vi "MDPtr PointerTotalCount.vi"(8 "error in (no error)":errorcluster) -> (0 "error out":errorcluster, 2 "MDPtr Total Count":i32)   [LabVIEW 2017, in "MDPtr.lvlib"]
uses:
  MDPtr.lvlib
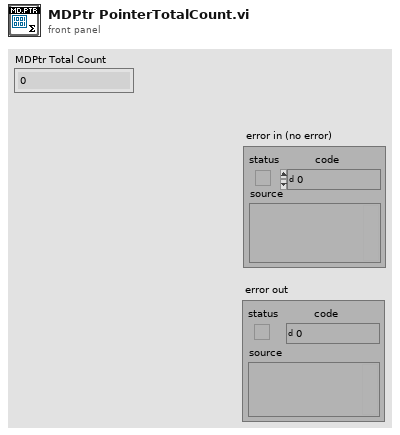
[diagram p1: front panel]
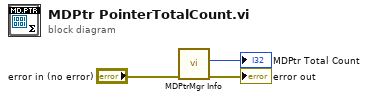
[diagram p0: block diagram]
diagram:
  n1 = call "MDPtrMgr Info.vi"("error in (no error)"="error in (no error)") -> ("error out"=→"error out":errorcluster, "# MDPtrs allocated"=→"MDPtr Total Count":i32)  [unwired: 6 in, 3 out]
